vi "Main Editor UI.vi"() -> ()   [LabVIEW 2015, in "E2E Tag Exchange editor node.lvclass"]
doc: "This is the main view for configuration the behavior of a module in the DCAF standard editor."
uses:
  E2E Tag Exchange editor node.lvclass
  <vilib>/NI/Configuration Framework/Node/NodeRef.ctl
  <vilib>/NI/Configuration Framework/Node/NISE_CEF_Node.lvclass
  <vilib>/NI/AMC/Message Queue.ctl
  <vilib>/NI/AMC/Message.ctl
  <vilib>/NI/Tools/Keyed Array/KeyedArray.ctl
  <vilib>/NI/Configuration Framework/Node/StopEvent.ctl
  <vilib>/NI/Configuration Framework/Node/RefreshUIEvent.ctl
  <vilib>/NI/Configuration Framework/Node/CacheState.ctl
  <vilib>/NI/Configuration Framework/Node/NodeChangeEvent.ctl
  <vilib>/NI/DCAF UI Toolkit/Controls/Move One Right.ctl
  <vilib>/NI/DCAF UI Toolkit/Controls/Move All Right.ctl
  <vilib>/NI/DCAF UI Toolkit/Controls/Move One Left.ctl
  <vilib>/NI/DCAF UI Toolkit/Controls/Move All Left.ctl
  module/configuration/Runtime Implementation.ctl
  references.ctl
  Pairing Tab References.ctl
  Tag Exchange Tab References.ctl
  <vilib>/Utility/miscctls.llb/LVPositionTypeDef.ctl
  <vilib>/NI/Tools/Keyed Array/Tools_KeyedArray.lvlib
  <vilib>/NI/AMC/AMC.lvlib
  <vilib>/NI/DCAF UI Toolkit/Controls/DCAF UI Elements.lvlib
  <vilib>/NI/DCAF/Tag Editor Core/Configuration Editor/Classes/Engine Parent/Engine Parent Editor Node.lvclass
  module/configuration/E2E Tag Exchange configuration.lvclass
panel:
  in  "node change":T1
  in  "cache state":T2
  in  "refresh UI":T3
  in  "stop event":T4
  in  "Tab Control":T5(tab)
  out "Paired Module UID":string
  in  "Unpair":bool
  in  "Pair":bool
  in  "implementation":T6 caption="Runtime Implementation"
  in  "E2E Nodes":i32(listbox)
  in  "Prefix":string
  out "From External Engine":i32(listbox)
  in  "To External Engine":i32(listbox)
  in  "Suffix":string
  in  "Move All Left":T7
  in  "Move One Left":T8
  in  "Move All Right":T9
  in  "Move One Right":T10
  in  "Filter":string
  in  "Available Tag List":i32(listbox)
  in  "main queue":T11
  in  "node ref":T12
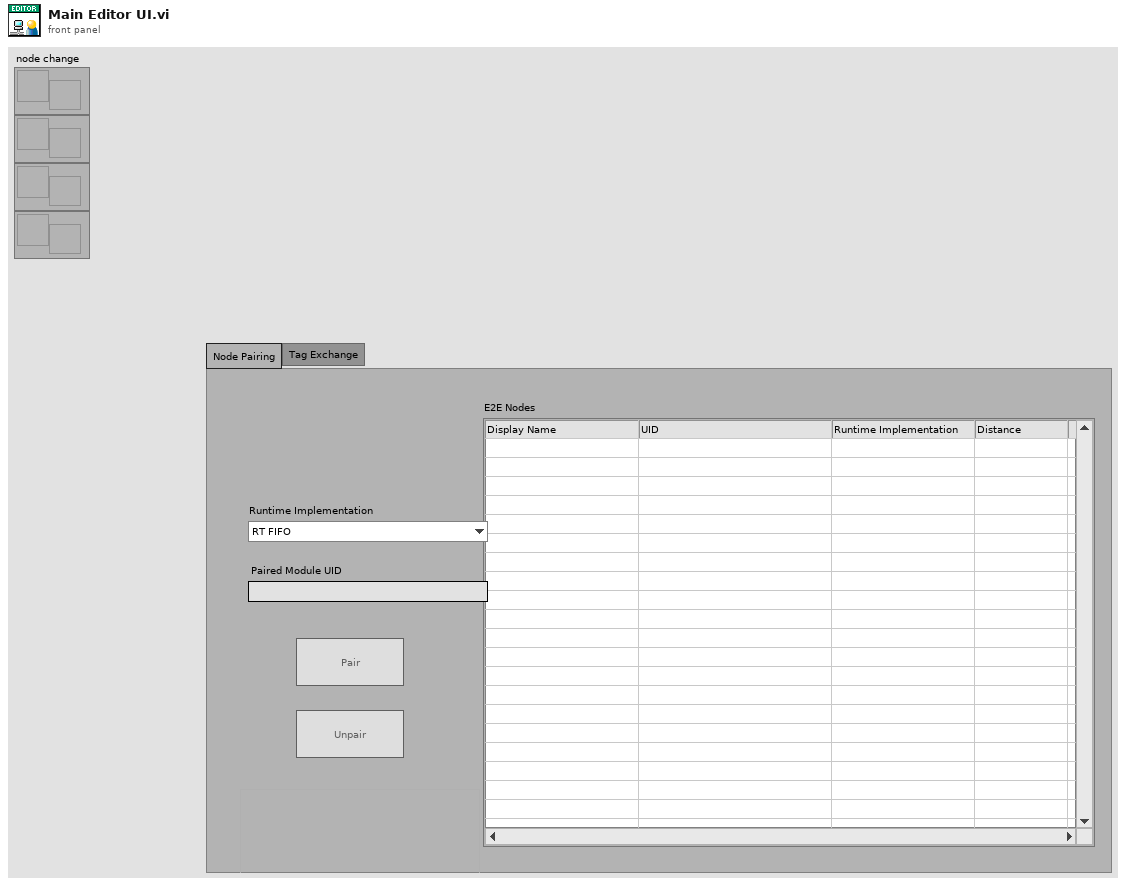
[diagram p1: front panel]
types:
  T1 = typedef "NISE_CEF_Node.lvclass/NodeChangeEvent.ctl" = refnum<user-event>
  T2 = typedef "NISE_CEF_Node.lvclass/CacheState.ctl" = refnum<user-event>
  T3 = typedef "NISE_CEF_Node.lvclass/RefreshUIEvent.ctl" = refnum<user-event>
  T4 = typedef "NISE_CEF_Node.lvclass/StopEvent.ctl" = refnum<user-event>
  T5 = enum32{"Node Pairing", "Tag Exchange", "Runtime Specific"}
  T6 = typedef "E2E Tag Exchange configuration.lvclass/Runtime Implementation.ctl" = enum16{"RT FIFO", "UDP"}
  T7 = typedef "DCAF UI Elements.lvlib/Move All Left.ctl" = bool
  T8 = typedef "DCAF UI Elements.lvlib/Move One Left.ctl" = bool
  T9 = typedef "DCAF UI Elements.lvlib/Move All Right.ctl" = bool
  T10 = typedef "DCAF UI Elements.lvlib/Move One Right.ctl" = bool
  T11 = typedef "AMC.lvlib/Message Queue.ctl" = refnum<queue>
  T12 = typedef "NISE_CEF_Node.lvclass/NodeRef.ctl" = refnum<data-value>
  T13 = typedef "E2E Tag Exchange editor node.lvclass/Tag Exchange Tab References.ctl" = cluster{"Available Tag List":refnum<vi>, "To External Engine":refnum<vi>, "From External Engine":refnum<vi>, "Move One Right":refnum<vi>, "Move All Right":refnum<vi>, "Move One Left":refnum<vi>, "Move All Left":refnum<vi>, "Tag Prefix":refnum<vi>, "Tag Suffix":refnum<vi>}
  T14 = typedef "E2E Tag Exchange editor node.lvclass/Pairing Tab References.ctl" = cluster{"E2E Nodes":refnum<vi>, "Pair":refnum<vi>, "Unpair":refnum<vi>, "implementation":refnum<vi>, "Paired Module UID":refnum<vi>}
  T15 = typedef "E2E Tag Exchange editor node.lvclass/references.ctl" = cluster{"stop event":T4, "refresh UI":T3, "cache state":T2, "node change":T1, "main queue":T11, "Refresh Pairing":refnum<user-event>, "Stop Subpanel":refnum<user-event>}
  T16 = typedef "LVPositionTypeDef.ctl" = cluster{"Left":i32, "Top":i32}
  T17 = typedef "E2E Tag Exchange editor node.lvclass/object references.ctl" = cluster{"engine":refnum<data-value>, "Node Ref":refnum<data-value>}
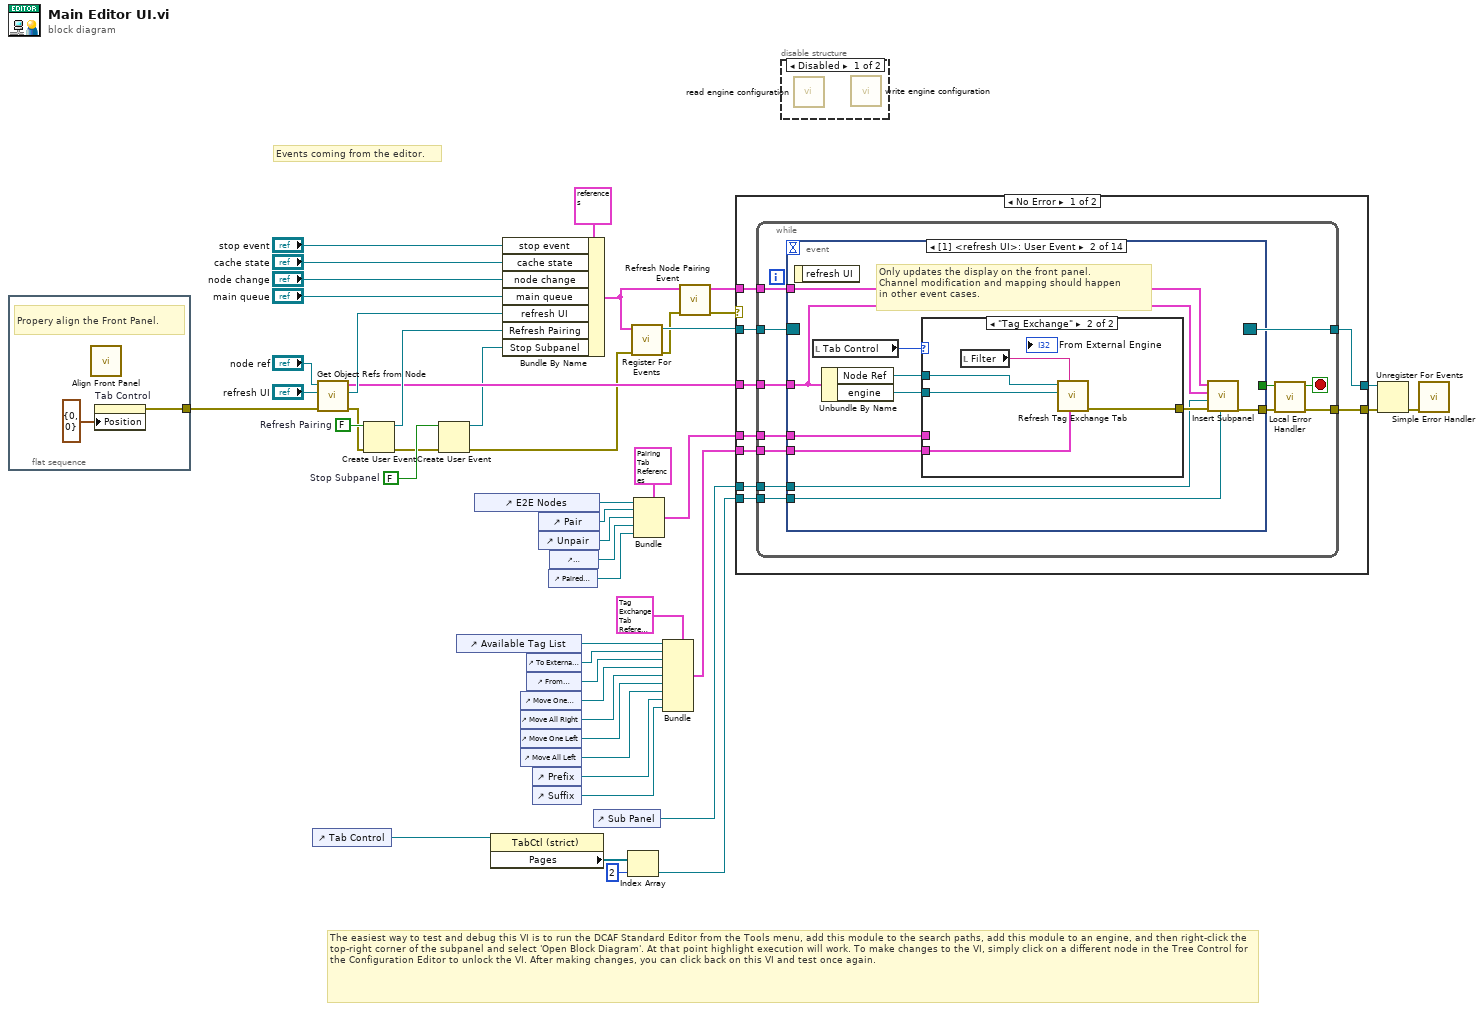
[diagram p0: block diagram]
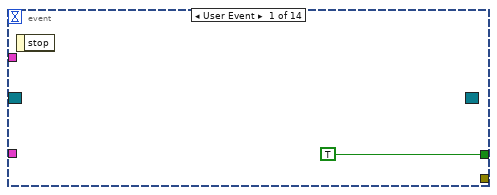
[diagram p3: hidden frame]
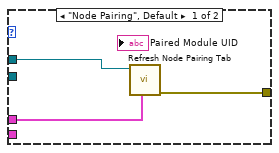
[diagram p4: hidden frame]
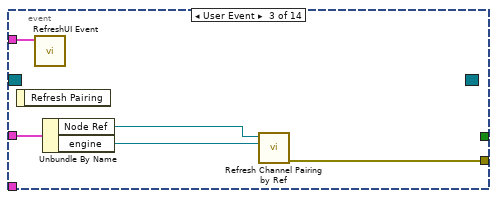
[diagram p5: hidden frame]
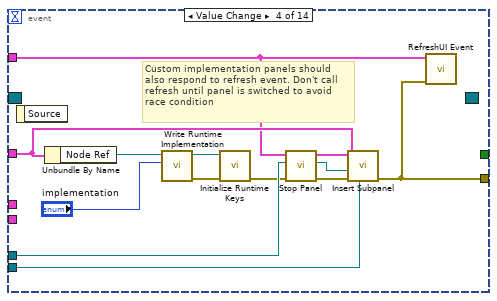
[diagram p6: hidden frame]
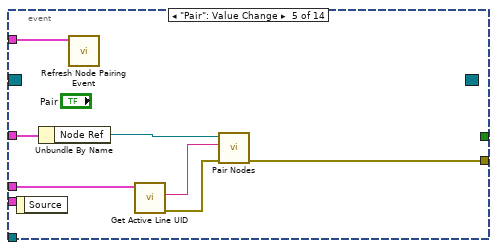
[diagram p7: hidden frame]
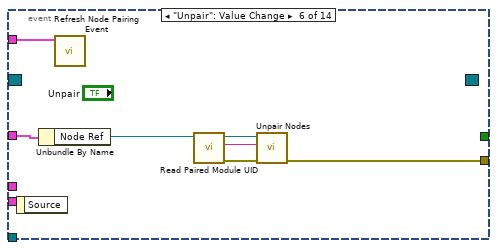
[diagram p8: hidden frame]
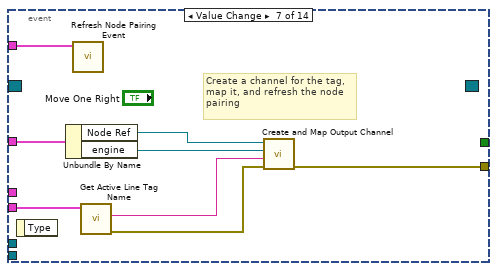
[diagram p9: hidden frame]
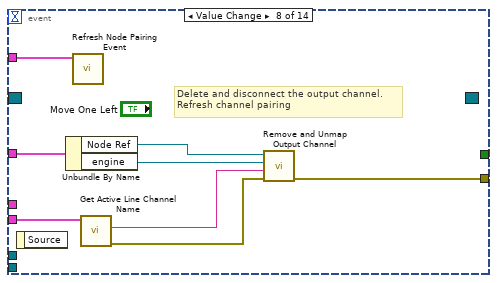
[diagram p10: hidden frame]
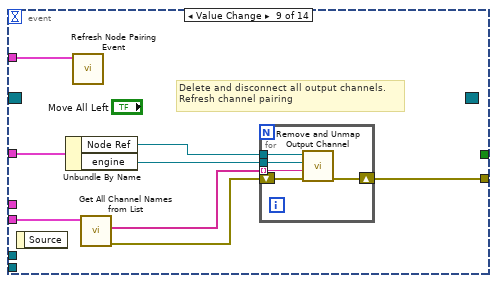
[diagram p11: hidden frame]
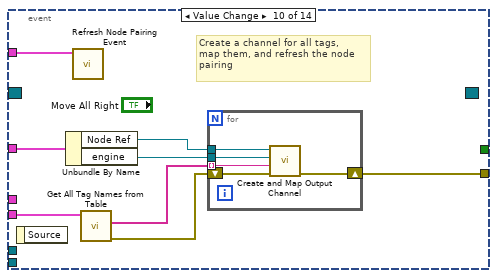
[diagram p12: hidden frame]
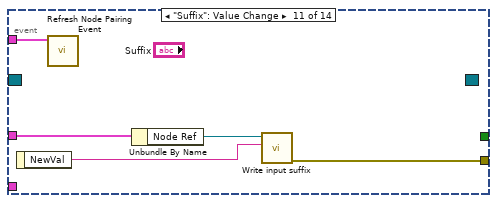
[diagram p13: hidden frame]
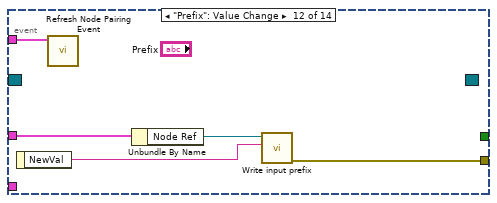
[diagram p14: hidden frame]
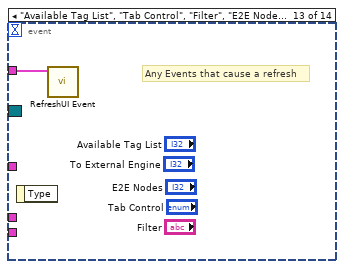
[diagram p15: hidden frame]
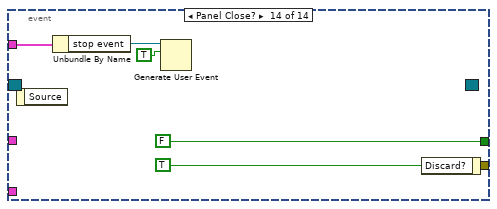
[diagram p16: hidden frame]
diagram:
  w5 = FALSE  # Stop Subpanel
  w31 = FALSE  # Refresh Pairing
  # "The easiest way to test and debug this VI is to run the DCAF Standard Editor from the Tools menu, add this module to the search paths, add this module to an engine, and then right-click the top-right corner of the subpanel and select 'Open Block Diagram'. At that point highlight execution will work. To make changes to the VI, simply click on a different node in the Tree Control for the Configuration Editor to unlock the VI. After making changes, you can click back on this VI and test once again."
  # "Events coming from the editor."
  n1 = flat-sequence {
    tunnel: [w49] -> w16
    frame #0 {
      # "Propery align the Front Panel."
      n2 = call <vilib>:"Align Front Panel.vi"() -> ()  [unwired: 10 in, 2 out]
      n3 = property on="Tab Control" class="TabCtl (strict)"("Position"=T16 {"Left"=0, "Top"=0}) -> (error out=w49:errorcluster)  [unwired: 2 in, 1 out]
    }
  }
  n4 = control-ref of="Tab Control"() -> (w9:refnum<vi>)
  n5 = call "Get Object Refs from Node.vi"("error in (no error)"=w16, "Refresh UI"="refresh UI", "Data Value Reference in"="node ref") -> ("error out"=w19:errorcluster, "Refresh UI out"=w37:T3, "References"=w17:T17)  [unwired: 6 in]
  n6 = Create User Event(user event datatype=w31, error in=w19) -> (user event=w18:refnum<user-event>, error out=w3:errorcluster)
  n7 = Create User Event(user event datatype=w5, error in=w3) -> (user event=w2:refnum<user-event>, error out=w1:errorcluster)
  n8 = control-ref of="Available Tag List"() -> (w28:refnum<vi>)
  n9 = control-ref of="E2E Nodes"() -> (w36:refnum<vi>)
  n10 = property class="TabCtl (strict)"(reference=w9) -> ("Pages"=w8:refnum<vi>[])  [unwired: 1 in, 2 out]
  n11 = Bundle By Name(cluster=T15 {"stop event"=refnum, "refresh UI"=refnum, "cache state"=refnum, "node change"=refnum, "main queue"=refnum, "Refresh Pairing"=refnum, "Stop Subpanel"=refnum} ("References"), "stop event"="stop event", "cache state"="cache state", "node change"="node change", "main queue"="main queue", "refresh UI"=w37, "Refresh Pairing"=w18, "Stop Subpanel"=w2) -> (w12:T15)
  n12 = control-ref of="Move One Right"() -> (w27:refnum<vi>)
  n13 = control-ref of="Move All Right"() -> (w26:refnum<vi>)
  n14 = control-ref of="Move One Left"() -> (w25:refnum<vi>)
  n15 = control-ref of="Move All Left"() -> (w24:refnum<vi>)
  n16 = control-ref of="To External Engine"() -> (w23:refnum<vi>)
  n17 = control-ref of="From External Engine"() -> (w22:refnum<vi>)
  n18 = control-ref of="Prefix"() -> (w15:refnum<vi>)
  n19 = control-ref of="Suffix"() -> (w14:refnum<vi>)
  n20 = control-ref of="Pair"() -> (w35:refnum<vi>)
  n21 = control-ref of="Unpair"() -> (w34:refnum<vi>)
  n22 = control-ref of="Paired Module UID"() -> (w29:refnum<vi>)
  n23 = control-ref of="implementation"() -> (w33:refnum<vi>)
  n24 = control-ref of="Sub Panel"() -> (w4:refnum<vi>)
  n25 = Index Array(array=w8, index=2) -> (element=w6:refnum<vi>)
  n26 = call "Register For Events.vi"("error in"=w1, "References"=w12) -> ("error out"=w11:errorcluster, "Event Registration Refnum"=w39:refnum<event-registration>)  [unwired: 8 in]
  n27 = Bundle(cluster=T14 {"E2E Nodes"=refnum, "Pair"=refnum, "Unpair"=refnum, "implementation"=refnum, "Paired Module UID"=refnum} ("Pairing Tab References"), "E2E Nodes"=w36, "Pair"=w35, "Unpair"=w34, "implementation"=w33, "Paired Module UID"=w29) -> (w30:T14)
  n28 = Bundle(cluster=T13 {"Available Tag List"=refnum, "To External Engine"=refnum, "From External Engine"=refnum, "Move One Right"=refnum, "Move All Right"=refnum, "Move One Left"=refnum, "Move All Left"=refnum, "Tag Prefix"=refnum, "Tag Suffix"=refnum} ("Tag Exchange Tab References"), "Available Tag List"=w28, "To External Engine"=w23, "From External Engine"=w22, "Move One Right"=w27, "Move All Right"=w26, "Move One Left"=w25, "Move All Left"=w24, "Tag Prefix"=w15, "Tag Suffix"=w14) -> (w20:T13)
  n29 = call "Refresh Node Pairing Event.vi"("error in (no error)"=w11, "References in"=w12) -> ("error out"=w10:errorcluster, "References out"=w13:T15)  [unwired: 8 in]
  n30 = case shown="No Error" w10 {
    selector: w10 -> [_ w183]
    tunnel: w39 -> [w59 w182]
    tunnel: [w58 w182] -> w48
    tunnel: [w55 w183] -> w47
    tunnel: w13 -> [w57 _]
    tunnel: w17 -> [w56 _]
    tunnel: w30 -> [w54 _]
    tunnel: w20 -> [w53 _]
    tunnel: w6 -> [w52 _]
    tunnel: w4 -> [w51 _]
    frame No Error {
      n31 = while {
        tunnel: w59 -> [w71]
        tunnel: [w70] -> w58
        tunnel: [w67] -> w55
        tunnel: w57 -> [w65]
        tunnel: w56 -> [w64]
        tunnel: w54 -> [w63]
        tunnel: w53 -> [w62]
        tunnel: w52 -> [w61]
        tunnel: w51 -> [w60]
        stop <- w69 stop-if-true
        n32 = event shown="[1] <refresh UI>: User Event" {
          selector: w71 -> [_ _ _ _ _ _ _ _ _ _ _ _ _ _]
          dyn-events: [_ _ _ _ _ _ _ _ _ _ _ _ _ _] -> w70
          timeout: _ -> [_ _ _ _ _ _ _ _ _ _ _ _ _ _]
          tunnel: [TRUE _ _ _ _ _ _ _ _ _ _ _ _ FALSE] -> w68
          tunnel: [_ w76 w94 w98 w115 w122 w127 w135 w143 w156 w169 w174 _ _] -> w66
          tunnel: w65 -> [_ w77 w95 w97 w110 w117 w124 w132 w140 w154 w166 w171 w176 w178]
          tunnel: w64 -> [_ w75 w96 w101 w116 w123 w130 w138 w146 w159 w170 w175 _ _]
          tunnel: w63 -> [_ w82 _ _ w112 _ _ _ _ _ _ _ _ _]
          tunnel: w62 -> [_ w79 _ _ _ _ w131 w139 w147 w160 _ _ _ _]
          tunnel: w61 -> [_ w73 _ w105 _ _ _ _ _ _ _ _ _ _]
          tunnel: w60 -> [_ w74 _ w106 _ _ _ _ _ _ _ _ _ _]
          event User Event {
            n33 = event-data() -> ()  [unwired: 1 in, 1 out]
          }
          event User Event {
            # "Only updates the display on the front panel.\nChannel modification and mapping should happen\nin other event cases."
            n34 = event-data() -> ()  [unwired: 1 in, 1 out]
            n35 = local read "Tab Control"() -> (w81:T5)
            n36 = Unbundle By Name(w75) -> ("Node Ref"=w83:refnum<data-value>, "engine"=w80:refnum<data-value>)
            n37 = case shown="\"Tag Exchange\"" w81 {
              tunnel: [w86 w89] -> w78
              tunnel: w83 -> [w84 w91]
              tunnel: w82 -> [w85 _]
              tunnel: w80 -> [_ w90]
              tunnel: w79 -> [_ w87]
              frame "Node Pairing", Default {
                n38 = call "Refresh Node Pairing Tab.vi"("Pairing Tab References"=w85, "E2E editor node in"=w84) -> ("error out"=w86:errorcluster)  [unwired: 8 in, 1 out]
              }
              frame "Tag Exchange" {
                n39 = local read "Filter"() -> (w88:string)
                n40 = call "Refresh Tag Exchange Tab.vi"("Tag Exchange Tab References"=w87, "Filter"=w88, "engine"=w90, "E2E editor node in"=w91) -> ("error out"=w89:errorcluster)  [unwired: 5 in, 2 out]
              }
            }
            n41 = call "Insert Subpanel.vi"("Page Refnum"=w73, "error in (no error)"=w78, "Subpanel reference"=w74, "node References"=w75, "References"=w77) -> ("error out"=w76:errorcluster)  [unwired: 6 in]
          }
          event User Event {
            n42 = event-data() -> ()  [unwired: 1 in, 1 out]
            n43 = call "RefreshUI Event.vi"("References in"=w95) -> ()  [unwired: 9 in, 2 out]
            n44 = Unbundle By Name(w96) -> ("Node Ref"=w92:refnum<data-value>, "engine"=w93:refnum<data-value>)
            n45 = call "Refresh Channel Pairing by Ref.vi"("engine"=w93, "E2E editor node in"=w92) -> ("error out"=w94:errorcluster)  [unwired: 7 in, 2 out]
          }
          event Value Change {
            # "Custom implementation panels should\nalso respond to refresh event. Don't call\nrefresh until panel is switched to avoid\nrace condition"
            n46 = event-data() -> ()  [unwired: 1 in, 1 out]
            n47 = Unbundle By Name(w101) -> ("Node Ref"=w109:refnum<data-value>)
            n48 = call "Write Runtime Implementation.vi"("Runtime Implementation"="implementation", "E2E editor node in"=w109) -> ("error out"=w102:errorcluster, "E2E editor node out"=w103:refnum<data-value>)  [unwired: 8 in]
            n49 = call "Initialize Runtime Keys.vi"("error in (no error)"=w102, "E2E editor node in"=w103) -> ("error out"=w99:errorcluster)  [unwired: 8 in, 1 out]
            n50 = call "Stop Panel.vi"("error in (no error)"=w99, "SubPanel reference"=w106, "References in"=w97) -> ("error out"=w107:errorcluster, "SubPanel reference out"=w100:refnum<vi>, "References out"=w108:T15)  [unwired: 6 in]
            n51 = call "Insert Subpanel.vi"("Page Refnum"=w105, "error in (no error)"=w107, "Subpanel reference"=w100, "node References"=w101, "References"=w108) -> ("error out"=w98:errorcluster)  [unwired: 6 in]
            n52 = call "RefreshUI Event.vi"("error in (no error)"=w98, "References in"=w97) -> ()  [unwired: 8 in, 2 out]
          }
          event "Pair": Value Change {
            n53 = event-data() -> ()  [unwired: 1 in, 1 out]
            n54 = Unbundle By Name(w116) -> ("Node Ref"=w114:refnum<data-value>)
            n55 = call "Refresh Node Pairing Event.vi"("References in"=w110) -> ()  [unwired: 9 in, 2 out]
            n56 = call "Get Active Line UID.vi"("Pairing Tab Refs"=w112) -> ("error out"=w113:errorcluster, "Line UID"=w111:string)  [unwired: 9 in]
            n57 = call "Pair Nodes.vi"("error in (no error)"=w113, "Node UID to Pair"=w111, "E2E editor node in"=w114) -> ("error out"=w115:errorcluster)  [unwired: 7 in, 1 out]
          }
          event "Unpair": Value Change {
            n58 = event-data() -> ()  [unwired: 1 in, 1 out]
            n59 = Unbundle By Name(w123) -> ("Node Ref"=w121:refnum<data-value>)
            n60 = call "Refresh Node Pairing Event.vi"("References in"=w117) -> ()  [unwired: 9 in, 2 out]
            n61 = call "Read Paired Module UID.vi"("E2E editor node in"=w121) -> ("error out"=w118:errorcluster, "Paired Module UID"=w119:string, "E2E editor node out"=w120:refnum<data-value>)  [unwired: 8 in]
            n62 = call "Unpair Nodes.vi"("error in (no error)"=w118, "Node UID to Unpair"=w119, "E2E editor node in"=w120) -> ("error out"=w122:errorcluster)  [unwired: 7 in, 1 out]
          }
          event Value Change {
            # "Create a channel for the tag,\nmap it, and refresh the node\npairing"
            n63 = event-data() -> ()  [unwired: 1 in, 1 out]
            n64 = Unbundle By Name(w130) -> ("Node Ref"=w128:refnum<data-value>, "engine"=w129:refnum<data-value>)
            n65 = call "Refresh Node Pairing Event.vi"("References in"=w124) -> ()  [unwired: 9 in, 2 out]
            n66 = call "Get Active Line Tag Name.vi"("Pairing Tab Refs"=w131) -> ("error out"=w126:errorcluster, "Tag Name"=w125:string)  [unwired: 9 in]
            n67 = call "Create and Map Output Channel.vi"("error in (no error)"=w126, "Tag Name"=w125, "engine"=w129, "E2E editor node in"=w128) -> ("error out"=w127:errorcluster)  [unwired: 5 in, 2 out]
          }
          event Value Change {
            # "Delete and disconnect the output channel.\nRefresh channel pairing"
            n68 = event-data() -> ()  [unwired: 1 in, 1 out]
            n69 = Unbundle By Name(w138) -> ("Node Ref"=w136:refnum<data-value>, "engine"=w137:refnum<data-value>)
            n70 = call "Refresh Node Pairing Event.vi"("References in"=w132) -> ()  [unwired: 9 in, 2 out]
            n71 = call "Get Active Line Channel Name.vi"("Pairing Tab Refs"=w139) -> ("error out"=w134:errorcluster, "Channel Name"=w133:string)  [unwired: 9 in]
            n72 = call "Remove and Unmap Output Channel.vi"("error in (no error)"=w134, "Channel Name"=w133, "engine"=w137, "E2E editor node in"=w136) -> ("error out"=w135:errorcluster)  [unwired: 5 in, 2 out]
          }
          event Value Change {
            # "Delete and disconnect all output channels.\nRefresh channel pairing"
            n73 = event-data() -> ()  [unwired: 1 in, 1 out]
            n74 = Unbundle By Name(w146) -> ("Node Ref"=w144:refnum<data-value>, "engine"=w145:refnum<data-value>)
            n75 = call "Refresh Node Pairing Event.vi"("References in"=w140) -> ()  [unwired: 9 in, 2 out]
            n76 = call "Get All Channel Names from List.vi"("Pairing Tab Refs"=w147) -> ("error out"=w142:errorcluster, "Channel Names"=w141:string[])  [unwired: 9 in]
            n77 = for {
              tunnel: w145 -> [w152]
              tunnel: w144 -> [w151]
              tunnel: w141 -> [w148] mode=indexing
              shift-right: [w150] -> w143
              shift-left: w142 -> [w149]
              n78 = call "Remove and Unmap Output Channel.vi"("error in (no error)"=w149, "Channel Name"=w148, "engine"=w152, "E2E editor node in"=w151) -> ("error out"=w150:errorcluster)  [unwired: 5 in, 2 out]
            }
          }
          event Value Change {
            # "Create a channel for all tags,\nmap them, and refresh the node\npairing"
            n79 = event-data() -> ()  [unwired: 1 in, 1 out]
            n80 = Unbundle By Name(w159) -> ("Node Ref"=w157:refnum<data-value>, "engine"=w158:refnum<data-value>)
            n81 = call "Refresh Node Pairing Event.vi"("References in"=w154) -> ()  [unwired: 9 in, 2 out]
            n82 = call "Get All Tag Names from Table.vi"("Pairing Tab Refs"=w160) -> ("error out"=w155:errorcluster, "Tag Names"=w153:string[])  [unwired: 9 in]
            n83 = for {
              tunnel: w158 -> [w165]
              tunnel: w157 -> [w164]
              shift-right: [w163] -> w156
              shift-left: w155 -> [w162]
              tunnel: w153 -> [w161] mode=indexing
              n84 = call "Create and Map Output Channel.vi"("error in (no error)"=w162, "Tag Name"=w161, "engine"=w165, "E2E editor node in"=w164) -> ("error out"=w163:errorcluster)  [unwired: 5 in, 2 out]
            }
          }
          event "Suffix": Value Change {
            n85 = event-data() -> ("NewVal"=w167:string)  [unwired: 1 in]
            n86 = call "Refresh Node Pairing Event.vi"("References in"=w166) -> ()  [unwired: 9 in, 2 out]
            n87 = Unbundle By Name(w170) -> ("Node Ref"=w168:refnum<data-value>)
            n88 = call "Write input suffix.vi"("Input Suffix"=w167, "E2E editor node in"=w168) -> ("error out"=w169:errorcluster)  [unwired: 8 in, 1 out]
          }
          event "Prefix": Value Change {
            n89 = event-data() -> ("NewVal"=w172:string)  [unwired: 1 in]
            n90 = call "Refresh Node Pairing Event.vi"("References in"=w171) -> ()  [unwired: 9 in, 2 out]
            n91 = Unbundle By Name(w175) -> ("Node Ref"=w173:refnum<data-value>)
            n92 = call "Write input prefix.vi"("Input Prefix"=w172, "E2E editor node in"=w173) -> ("error out"=w174:errorcluster)  [unwired: 8 in, 1 out]
          }
          event "Available Tag List", "Tab Control", "Filter", "E2E Nodes", "To External Engine": Value Change {
            # "Any Events that cause a refresh"
            n93 = event-data() -> ()  [unwired: 1 in, 1 out]
            n94 = call "RefreshUI Event.vi"("References in"=w176) -> ()  [unwired: 9 in, 2 out]
          }
          event Panel Close? {
            n95 = event-data() -> ()  [unwired: 1 in, 1 out]
            n96 = Unbundle By Name(w178) -> ("stop event"=w177:T4)
            n97 = Generate User Event(user event=w177, event data cluster=TRUE ("event data")) -> ()  [unwired: 2 in, 2 out]
            n98 = event-data("Discard?"=TRUE) -> ()  [unwired: 1 in, 1 out]
          }
        }
        n99 = call "Local Error Handler.vi"("error in"=w66, "Stop in"=w68) -> ("error out"=w67:errorcluster, "Stop out"=w69:bool)  [unwired: 8 in]
      }
    }
    frame Error {
    }
  }
  n100 = disable-structure shown="Disabled" {
    frame Disabled {
      n101 = call <vilib>:"read engine configuration.vi"() -> ()  [unwired: 9 in, 3 out]
      n102 = call <vilib>:"write engine configuration.vi"() -> ()  [unwired: 10 in, 2 out]
    }
    frame Enabled {
    }
  }
  n103 = Unregister For Events(event registration refnum=w48, error in=w47) -> (error out=w46:errorcluster)
  n104 = call <vilib>:"Simple Error Handler.vi"("error in (no error)"=w46) -> ()  [unwired: 4 in, 5 out]
